vi "Relative Colon Path.vi"(11 "error in":errorcluster) -> (4 "path text":string, 15 "error out":errorcluster)   [LabVIEW 2024]
doc: "Tests a relative path component containing a colon without accessing a file."
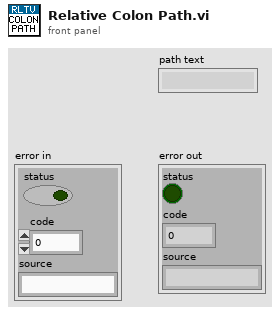
[diagram p1: front panel]
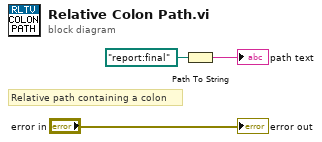
[diagram p0: block diagram]
diagram:
  # "Relative path containing a colon"
  n1 = Path To String(path=path "report:final" ("relative colon path")) -> (string=→"path text":string)
  "error out" <- "error in"
